vi "Ard_Wait_ms.vi"(8 "error in":errorcluster, 10 "millisec":u32) -> (0 "error in 2":errorcluster)   [LabVIEW 2021]
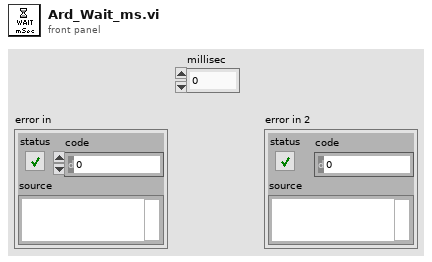
[diagram p1: front panel]
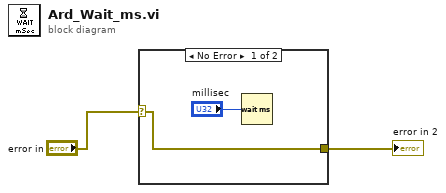
[diagram p0: block diagram]
diagram:
  n1 = case shown="No Error" "error in" {
    selector: "error in" -> [w3 w5]
    tunnel: [w3 w5] -> w1
    frame No Error {
      n2 = Wait (ms)(milliseconds to wait="millisec") -> ()  [unwired: 1 out]
    }
    frame Error {
    }
  }
  "error in 2" <- w1
